vi "recibe.vi"() -> ()   [LabVIEW 2017]
uses:
  <vilib>/Instr/_visa.llb/VISA Configure Serial Port (Instr).vi
panel:
  out "read buffer":string
  in  "stop":bool
  in  "PUERTO":refnum<visa-resource-name>
  in  "parar":bool
  in  "derecha":bool
  in  "izquierda":bool
  out "SUICHE":bool
  out "TEMPERATURA":dbl(slide) scale=0.0..100.0
  in  "VELOCIDAD":dbl(knob) scale=0.0..100.0
  in  "LED2":bool
  in  "LED1":bool
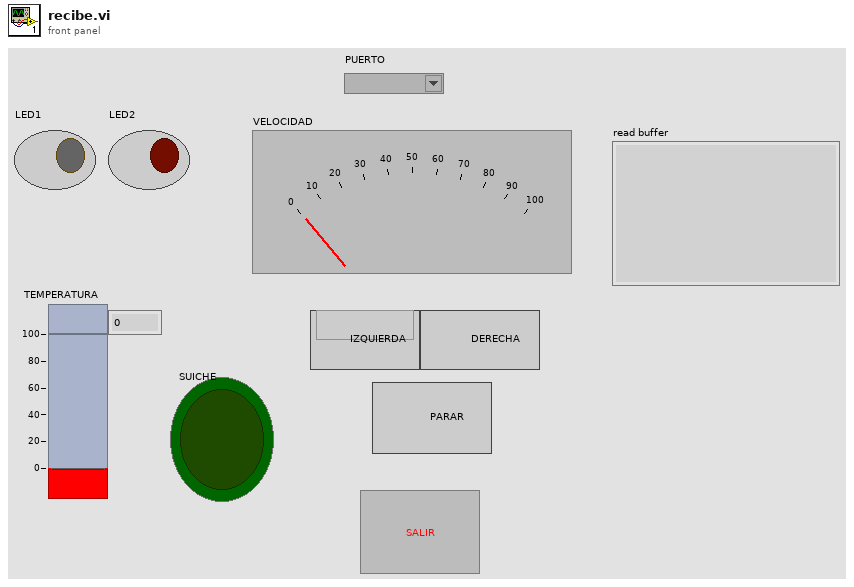
[diagram p1: front panel]
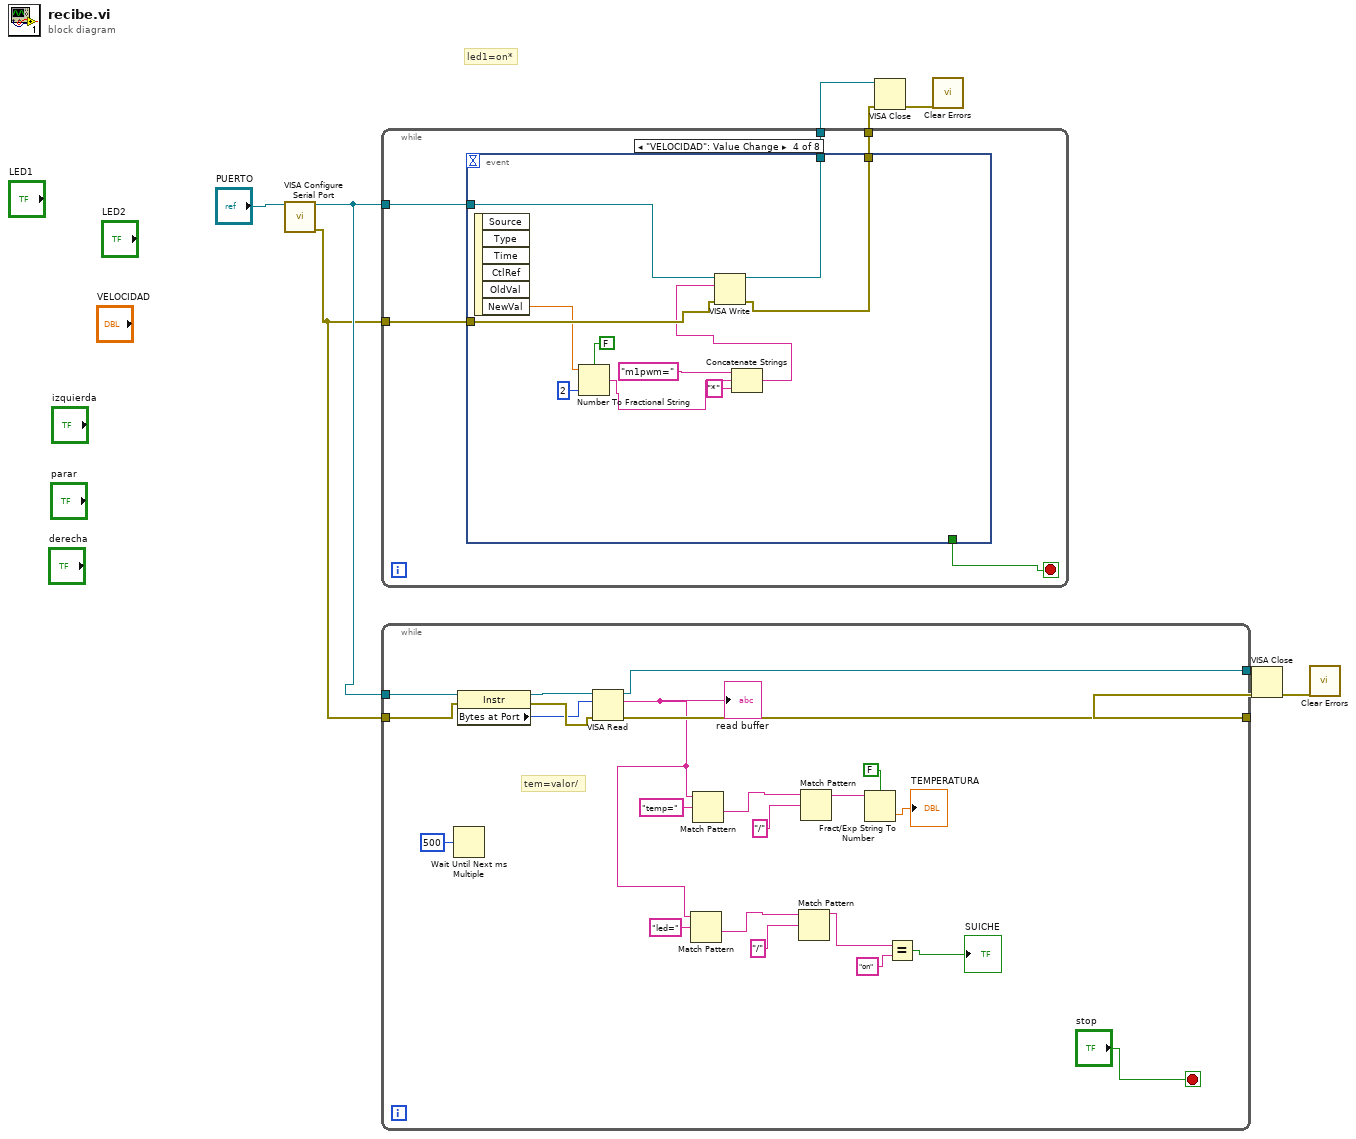
[diagram p0: block diagram]
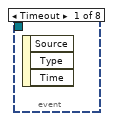
[diagram p2: hidden frame]
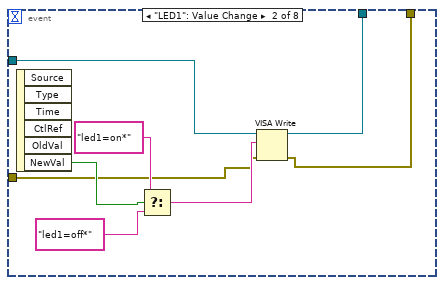
[diagram p3: hidden frame]
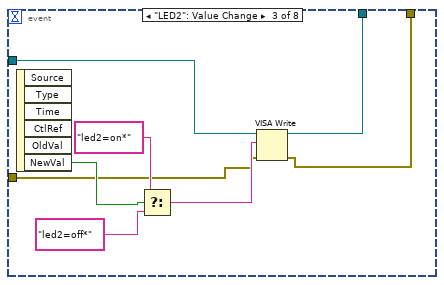
[diagram p4: hidden frame]
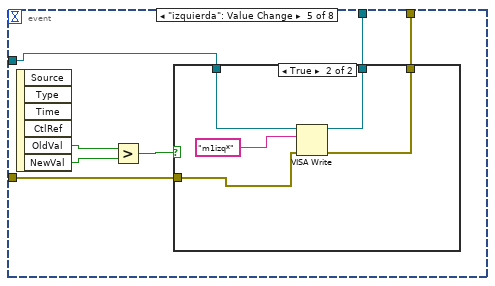
[diagram p5: hidden frame]
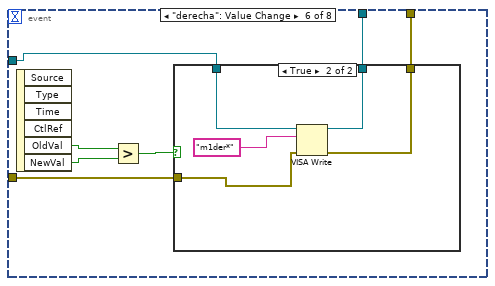
[diagram p7: hidden frame]
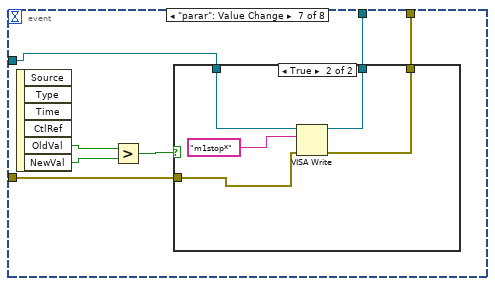
[diagram p9: hidden frame]
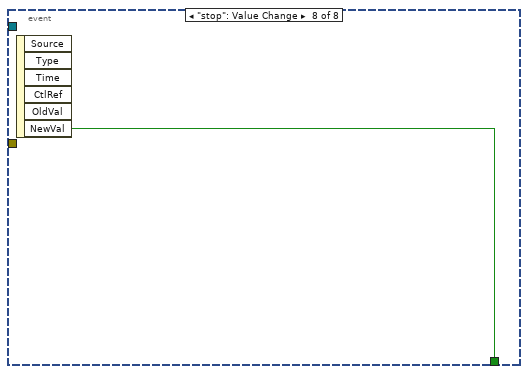
[diagram p11: hidden frame]
diagram:
  # "led1=on*"
  n1 = call-poly "VISA Configure Serial Port"("VISA resource name"="PUERTO") -> ("VISA resource name out"=w5:refnum<visa-resource-name>, "error out"=w4:errorcluster)  [unwired: 13 in]
  n2 = while {
    tunnel: w5 -> [w14]
    tunnel: w4 -> [w13]
    tunnel: [w12] -> w8
    tunnel: [w11] -> w7
    stop <- w10 stop-if-true
    n3 = event shown="[3] \"VELOCIDAD\": Value Change" {
      selector: _ -> [_ _ _ _ _ _ _ _]
      dyn-events: _ -> [_ _ _ _ _ _ _ _]
      timeout: _ -> [_ _ _ _ _ _ _ _]
      tunnel: w14 -> [_ w18 w26 w41 w45 w57 w69 _]
      tunnel: w13 -> [_ w17 w25 w40 w44 w56 w68 _]
      tunnel: [_ w16 w24 w39 w43 w55 w67 _] -> w12
      tunnel: [_ w15 w23 w38 w42 w54 w66 _] -> w11
      tunnel: [_ _ _ _ _ _ _ w78] -> w10
      event Timeout {
        n4 = event-data() -> ()  [unwired: 1 in, 3 out]
      }
      event "LED1": Value Change {
        n5 = event-data() -> ("NewVal"=w22:bool)  [unwired: 1 in, 5 out]
        n6 = Select(t="led1=on*", s=w22, f="led1=off*") -> (s? t:f=w19:string)
        n7 = VISA Write(VISA resource name=w18, write buffer=w19, error in (no error)=w17) -> (VISA resource name out=w16:refnum<visa-resource-name>, error out=w15:errorcluster)  [unwired: 1 out]
      }
      event "LED2": Value Change {
        n8 = event-data() -> ("NewVal"=w30:bool)  [unwired: 1 in, 5 out]
        n9 = Select(t="led2=on*", s=w30, f="led2=off*") -> (s? t:f=w27:string)
        n10 = VISA Write(VISA resource name=w26, write buffer=w27, error in (no error)=w25) -> (VISA resource name out=w24:refnum<visa-resource-name>, error out=w23:errorcluster)  [unwired: 1 out]
      }
      event "VELOCIDAD": Value Change {
        n11 = event-data() -> ("NewVal"=w37:dbl)  [unwired: 1 in, 5 out]
        n12 = Number To Fractional String(use system decimal point (T)=FALSE, number=w37, precision (6)=i16 2) -> (F-format string=w34:string)  [unwired: 1 in]
        n13 = Concatenate Strings("m1pwm=" ("string"), w34, "*" ("string")) -> (w32:string)
        n14 = VISA Write(VISA resource name=w41, write buffer=w32, error in (no error)=w40) -> (VISA resource name out=w39:refnum<visa-resource-name>, error out=w38:errorcluster)  [unwired: 1 out]
      }
      event "izquierda": Value Change {
        n15 = event-data() -> ("OldVal"=w48:bool, "NewVal"=w47:bool)  [unwired: 1 in, 4 out]
        n16 = Greater?(x=w48, y=w47) -> (0:w46:bool)
        n17 = case shown="True" w46 {
          tunnel: w45 -> [_ w53]
          tunnel: w44 -> [_ w52]
          tunnel: [_ w50] -> w43
          tunnel: [_ w49] -> w42
          frame False {
          }
          frame True {
            n18 = VISA Write(VISA resource name=w53, write buffer="m1izq*", error in (no error)=w52) -> (VISA resource name out=w50:refnum<visa-resource-name>, error out=w49:errorcluster)  [unwired: 1 out]
          }
        }
      }
      event "derecha": Value Change {
        n19 = event-data() -> ("OldVal"=w60:bool, "NewVal"=w59:bool)  [unwired: 1 in, 4 out]
        n20 = Greater?(x=w60, y=w59) -> (0:w58:bool)
        n21 = case shown="True" w58 {
          tunnel: w57 -> [_ w65]
          tunnel: w56 -> [_ w64]
          tunnel: [_ w62] -> w55
          tunnel: [_ w61] -> w54
          frame False {
          }
          frame True {
            n22 = VISA Write(VISA resource name=w65, write buffer="m1der*", error in (no error)=w64) -> (VISA resource name out=w62:refnum<visa-resource-name>, error out=w61:errorcluster)  [unwired: 1 out]
          }
        }
      }
      event "parar": Value Change {
        n23 = event-data() -> ("OldVal"=w72:bool, "NewVal"=w71:bool)  [unwired: 1 in, 4 out]
        n24 = Greater?(x=w72, y=w71) -> (0:w70:bool)
        n25 = case shown="True" w70 {
          tunnel: w69 -> [_ w77]
          tunnel: w68 -> [_ w76]
          tunnel: [_ w74] -> w67
          tunnel: [_ w73] -> w66
          frame False {
          }
          frame True {
            n26 = VISA Write(VISA resource name=w77, write buffer="m1stop*", error in (no error)=w76) -> (VISA resource name out=w74:refnum<visa-resource-name>, error out=w73:errorcluster)  [unwired: 1 out]
          }
        }
      }
      event "stop": Value Change {
        n27 = event-data() -> ("NewVal"=w78:bool)  [unwired: 1 in, 5 out]
      }
    }
  }
  n28 = while {
    tunnel: w5 -> [w95]
    tunnel: w4 -> [w94]
    tunnel: [w93] -> w2
    tunnel: [w92] -> w1
    stop <- "stop" stop-if-true
    # "tem=valor/"
    n29 = Wait Until Next ms Multiple(millisecond multiple=u32 500) -> ()  [unwired: 1 out]
    n30 = property class="Instr"(reference=w95, error in=w94) -> (reference out=w98:refnum<visa-resource-name>, error out=w97:errorcluster, "Bytes at Port"=w96:u32)
    n31 = VISA Read(VISA resource name=w98, byte count=w96, error in (no error)=w97) -> (VISA resource name out=w93:refnum<visa-resource-name>, read buffer=w82:string, error out=w92:errorcluster)  [unwired: 1 out]
    "read buffer" <- w82
    n32 = Match Pattern(string=w82, regular expression="led=") -> (after substring=w84:string)  [unwired: 1 in, 3 out]
    n33 = Match Pattern(string=w82, regular expression="temp=") -> (after substring=w90:string)  [unwired: 1 in, 3 out]
    n34 = Match Pattern(string=w84, regular expression="/") -> (before substring=w81:string)  [unwired: 1 in, 3 out]
    n35 = Match Pattern(string=w90, regular expression="/") -> (before substring=w88:string)  [unwired: 1 in, 3 out]
    n36 = Fract/Exp String To Number(use system decimal point (T)=FALSE, string=w88) -> (number=→"TEMPERATURA":dbl)  [unwired: 2 in, 1 out]
    n37 = Equal?(x=w81, y="on") -> (x = y?=→"SUICHE":bool)
  }
  n38 = VISA Close(VISA resource name=w8, error in (no error)=w7) -> (error out=w6:errorcluster)
  n39 = call <vilib>:"Clear Errors.vi"("error in (no error)"=w6) -> ()  [unwired: 5 in, 2 out]
  n40 = VISA Close(VISA resource name=w2, error in (no error)=w1) -> (error out=w3:errorcluster)
  n41 = call <vilib>:"Clear Errors.vi"("error in (no error)"=w3) -> ()  [unwired: 5 in, 2 out]
